vi "Valid Input Response.vi"(8 "error in":errorcluster, 10 "given?":bool, 11 "response":string) -> (0 "error out":errorcluster, 3 "valid?":bool)   [LabVIEW 2020, in "MCP Server.lvlib"]
doc: "Tells Ask User.vi whether the entry the client sent for a question in params.inputResponses is an answer.\n\nMCP 2026-07-28 says a server should validate inputResponses and ask again for input that is missing or invalid. valid? is TRUE only when given? is TRUE, response is a JSON object and its item action is exactly the string accept, decline or cancel. Everything else, for example 42, \"accept\" (a string instead of an object), {} or {\"action\":\"maybe\"}, is not an answer: Ask User.vi then treats the question as not answered and asks it again.\n\nThe content of an accepted answer is not checked against the requestedSchema; that is left to the tool VI. error in is passed to error out and does not change the result."
uses:
  MCP Server.lvlib
  <vilib>/JDP Science/JSONtext/Next JSON Value.vi
  <vilib>/JDP Science/JSONtext/String Subset.vi
  <vilib>/JDP Science/JSONtext/Parsing/Advance past next JSON Value (inlined COPY).vi
  <vilib>/JDP Science/JSONtext/Parsing/Advance past whitespace.vi
  <vilib>/JDP Science/JSONtext/Parsing/Advance past String.vi
  <vilib>/JDP Science/JSONtext/Parsing/Advance past Number.vi
  <vilib>/JDP Science/JSONtext/Parsing/Advance past Line Ending.vi
  <vilib>/JDP Science/JSONtext/Parsing/Parse Full Path or Item Name.vi
  <vilib>/JDP Science/JSONtext/Parsing/Advance past Array.vi
  <vilib>/JDP Science/JSONtext/Parsing/Advance past Object.vi
  <vilib>/JDP Science/JSONtext/support/Error Cluster From Code.vi
  <vilib>/JDP Science/JSONtext/Offset/Find Item Locations by Path.vi
  <vilib>/JDP Science/JSONtext/JSONtext.lvlib
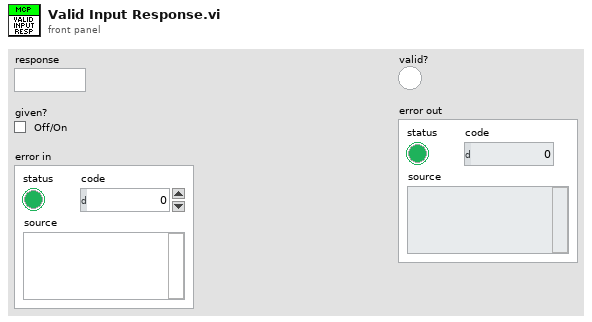
[diagram p1: front panel]
types:
  T1 = typedef "JSONtext.lvlib/JSON Value Type.ctl" = enum16{"Not a JSON Value", "JSON Object", "JSON Array", "String", "Number", "true", "false", "null"}
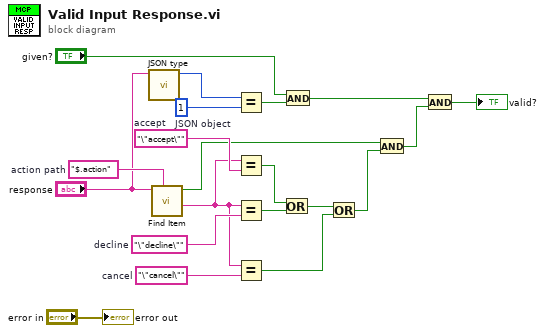
[diagram p0: block diagram]
diagram:
  w13 = "\"cancel\""  # cancel
  w15 = "\"decline\""  # decline
  w16 = "\"accept\""  # accept
  w18 = "$.action"  # action path
  w19 = u16 1  # JSON object
  n1 = call <vilib>:"JSON type.vi"("JSON"="response") -> ("JSON Value Type"=w20:T1)  [unwired: 9 in, 1 out]
  n2 = call <vilib>:"Find Item.vi"("$Path or Item Name"=w18, "JSON"="response") -> ("<JSON>"=w14:string, "Found"=w6:bool)  [unwired: 6 in, 2 out]
  n3 = Equal?(x=w20, y=w19) -> (x = y?=w7:bool)
  n4 = Equal?(x=w14, y=w16) -> (x = y?=w12:bool)
  n5 = Equal?(x=w14, y=w15) -> (x = y?=w11:bool)
  n6 = Equal?(x=w14, y=w13) -> (x = y?=w9:bool)
  n7 = Or(x=w12, y=w11) -> (x .or. y?=w10:bool)
  n8 = And(x="given?", y=w7) -> (x .and. y?=w4:bool)
  n9 = Or(x=w10, y=w9) -> (x .or. y?=w5:bool)
  n10 = And(x=w6, y=w5) -> (x .and. y?=w3:bool)
  n11 = And(x=w4, y=w3) -> (x .and. y?=→"valid?":bool)
  "error out" <- "error in"
